vi "Stream WaitEvent.vi"(8 "error in (no error)":errorcluster, 10 "Event":refnum<class "Event.lvclass">, 11 "Stream in":refnum<class "Stream.lvclass">) -> (0 "error out":errorcluster, 3 "Stream out":refnum<class "Stream.lvclass">)   [LabVIEW 2020, in "OpenLvVision_OpenCv.lvlib" / "Cuda.lvlib" / "Stream.lvclass"]
doc: "Instructs this GPU Stream to pause its execution until a specific CUDA Event triggers."
uses:
  Stream.lvclass
  OpenLvVision_OpenCv.lvlib
  _LvHelpers/EdvrObject/EdvrObject.lvclass
  <vilib>/Utility/error.llb/Error Cluster From Error Code.vi
  <vilib>/ErrorRing/Error Ring.xnode
  Dlls/OlvOpenCvWrapper.dll
  Event/Event.lvclass
  C:/Users/lukas/Downloads/OpenLvVision_OpenCv/SourceCode/LabView/OpenLvVision_OpenCv/_LvHelpers/EdvrObject/EdvrObject.lvclass
  C:/Users/lukas/Downloads/OpenLvVision_OpenCv/SourceCode/LabView/OpenLvVision_OpenCv/Cuda/DataAccess/Event/Event.lvclass
  C:/Users/lukas/Downloads/OpenLvVision_OpenCv/SourceCode/LabView/OpenLvVision_OpenCv/Cuda/DataAccess/Stream/Stream.lvclass
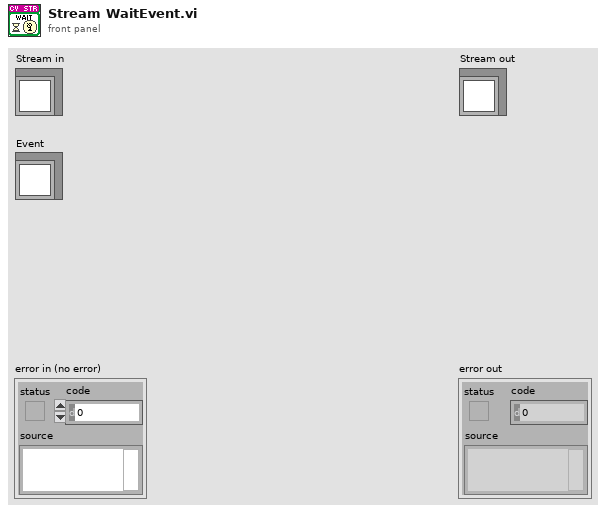
[diagram p1: front panel]
types:
  T1 = typedef "OpenLvVision_OpenCv.lvlib/EdvrObject.lvclass/Edvr.ctl" = refnum<data-value>
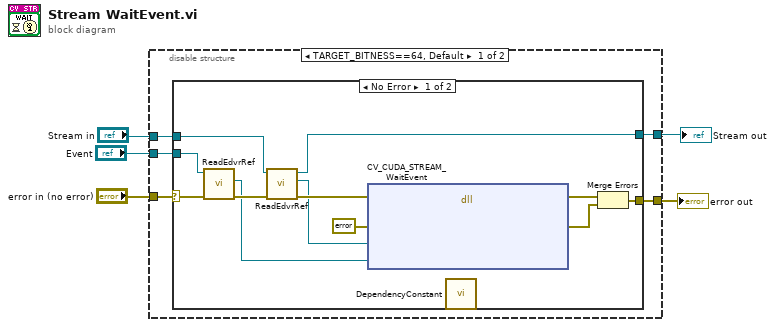
[diagram p0: block diagram]
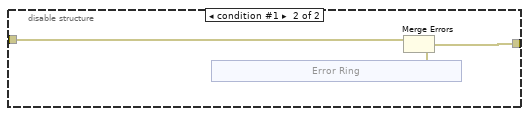
[diagram p3: hidden frame]
diagram:
  n1 = disable-structure shown="TARGET_BITNESS==64, Default" {
    disable-tunnel: "error in (no error)" -> [w7 w26]
    disable-tunnel: [w10 w27] -> w3
    disable-tunnel: [w9 _] -> w2
    disable-tunnel: "Stream in" -> [w8 _]
    disable-tunnel: "Event" -> [w6 _]
    frame condition #0 (active) {
      n2 = case shown="No Error" w7 {
        selector: w7 -> [w14 w24]
        tunnel: [w18 w24] -> w10
        tunnel: [w19 w23] -> w9
        tunnel: w8 -> [w17 w23]
        tunnel: w6 -> [w13 _]
        frame No Error {
          n3 = call "ReadEdvrRef.vi"("error in (no error)"=w14, "EdvrObject in"=w13) -> ("error out"=w12:errorcluster, "Edvr"=w11:T1)  [unwired: 7 in, 1 out]
          n4 = call "ReadEdvrRef.vi"("error in (no error)"=w12, "EdvrObject in"=w17) -> ("error out"=w21:errorcluster, "Edvr"=w20:T1, "EdvrObject out"=w19:refnum<class "Stream.lvclass">)  [unwired: 7 in]
          n5 = dll-call lib="C:/Users/lukas/Downloads/OpenLvVision_OpenCv/SourceCode/LabView/OpenLvVision_OpenCv/Dlls/OlvOpenCvWrapper.dll" fn="CV_CUDA_STREAM_WaitEvent"(error in=w21, "Error"=errorcluster {"status"=FALSE, "code"=0, "source"=""} ("error out"), "StreamEdvrRef"=w20, "EventEdvrRef"=w11) -> (error out=w15:errorcluster, "Error"=w16:errorcluster)  [unwired: 5 in, 1 out]
          n6 = call "DependencyConstant.vi"() -> ()  [unwired: 12 in]
          n7 = Merge Errors(w15, w16) -> (w18:errorcluster)
        }
        frame Error {
        }
      }
    }
    frame condition #1 {
      n8 = xnode "Error Ring"() -> ("error out"=w25:errorcluster)
      n9 = Merge Errors(w26, w25) -> (w27:errorcluster)
    }
  }
  "error out" <- w3
  "Stream out" <- w2
